vi "TCP Safe Read.vi"(8 "error in (no error)":errorcluster, 9 "timeout ms (25000)":i32, 10 "bytes to read":i32, 11 "TCP Network Connection in":refnum<k5>) -> (0 "error out":errorcluster, 2 "String":string, 3 "TCP Network Connection out":refnum<k5>)   [LabVIEW 2020, in "CSM-TCP-Router.lvlib"]
uses:
  CSM-TCP-Router.lvlib
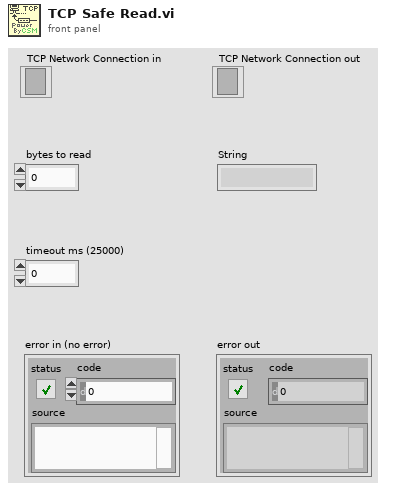
[diagram p1: front panel]
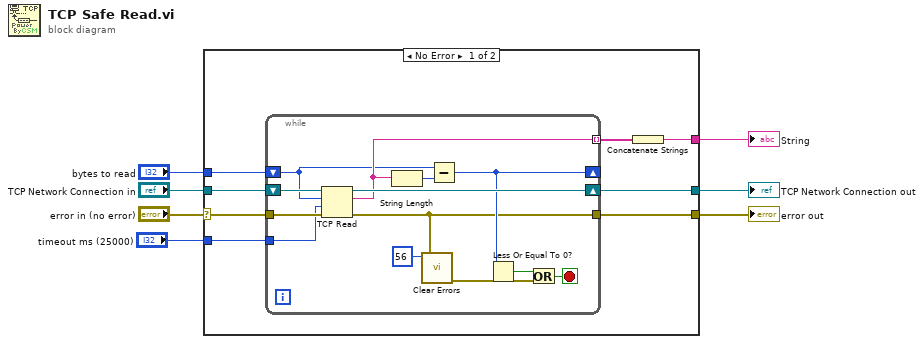
[diagram p0: block diagram]
diagram:
  n1 = case shown="No Error" "error in (no error)" {
    selector: "error in (no error)" -> [w10 w30]
    tunnel: [w15 _] -> w7
    tunnel: [w14 w30] -> w6
    tunnel: "bytes to read" -> [w12 _]
    tunnel: [w11 w29] -> w4
    tunnel: "TCP Network Connection in" -> [w9 w29]
    tunnel: "timeout ms (25000)" -> [w8 _]
    frame No Error {
      n2 = while {
        tunnel: [w25] -> w13 mode=indexing
        shift-right: [w26] -> w11
        shift-left: w9 -> [w28]
        shift-right: [w22] -> _
        shift-left: w12 -> [w23]
        tunnel: w8 -> [w20]
        tunnel: w10 -> [w27]
        tunnel: [w16] -> w14
        stop <- w18 stop-if-true
        n3 = TCP Read(connection ID=w28, bytes to read=w23, error in (no error)=w27, 9:w20) -> (connection ID out=w26:refnum<k5>, data out=w25:string, error out=w16:errorcluster)  [unwired: 1 in]
        n4 = String Length(string=w25) -> (length=w24:i32)
        n5 = call <vilib>:"Clear Errors.vi"("error in (no error)"=w16, "specific error code to clear (0: all)"=56) -> ("error out"=w17:errorcluster)  [unwired: 4 in, 1 out]
        n6 = Subtract(x=w23, y=w24) -> (x-y=w22:i32)
        n7 = Less Or Equal To 0?(x=w22) -> (x <= 0?=w21:bool)
        n8 = Or(x=w21, y=w17) -> (x .or. y?=w18:bool)
      }
      n9 = Concatenate Strings(w13) -> (w15:string)
    }
    frame Error {
    }
  }
  "String" <- w7
  "error out" <- w6
  "TCP Network Connection out" <- w4
